vi "Main.vi"(6 "Folder names":string[](array[string])=["StaARx#[PLC]StaATesterRxSignals", "StaATx#[PLC]StaATesterTxSignals"], 8 "error in":errorcluster, 9 "Sequence Context":refnum<k7>, 11 "OPC UA In":refnum<class "Abstract.lvclass">=refnum) -> (0 "error out":errorcluster, 3 "OPC UA Out":refnum<class "Abstract.lvclass">)   [LabVIEW 2025, in "Abstract.lvclass"]
uses:
  Abstract.lvclass
  Tester Rx Dataset.ctl
  Tester Tx Dataset.ctl
  Abstract.lvclass/Abstract.ctl
  Read OPC UA Ref.vi
  Write Rx from PLC.vi
  Write Tx to PLC.vi
  Write Subscription.vi
  <vilib>/OPCUA/NI OPC UA Client.lvlib
panel:
  in  "Tx to PLC":T1
  out "Rx from PLC":T2={"Start"=FALSE, "NestStatus"=FALSE, "PalletID"=0, "BarcodeData"="P:10-000001R:04S:QMC2200001", "StepEcho"=0, "Cylinder_1"=FALSE, "Cylinder_2"=FALSE, "Cylinder_3"=FALSE, "Cylinder_4"=FALSE, "Cylinder_5"=FALSE, "ResultsAck"=FALSE, "Reset"=FALSE, "Stop"=FALSE, "FaultCode"=0}
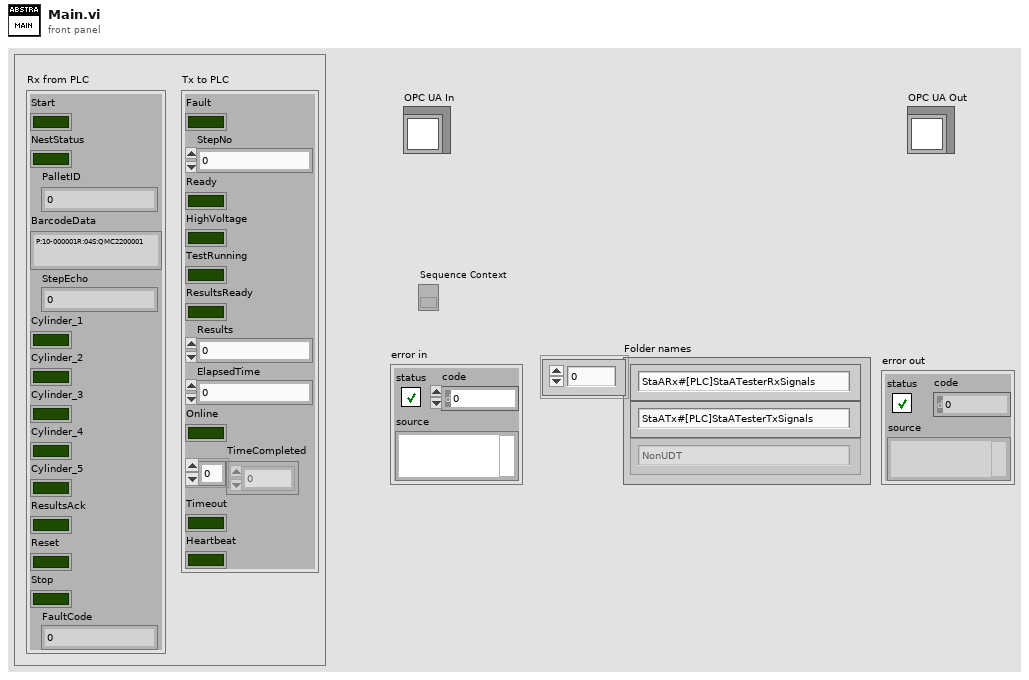
[diagram p1: front panel]
types:
  T1 = typedef "Abstract.lvclass/Tester Tx Dataset.ctl" = cluster{"Fault":bool, "StepNo":u32, "Ready":bool, "HighVoltage":bool, "TestRunning":bool, "ResultsReady":bool, "Results":u32, "ElapsedTime":u32, "Online":bool, "TimeCompleted":i32[], "Timeout":bool, "Heartbeat":bool}
  T2 = typedef "Abstract.lvclass/Tester Rx Dataset.ctl" = cluster{"Start":bool, "NestStatus":bool, "PalletID":u32, "BarcodeData":string, "StepEcho":u32, "Cylinder_1":bool, "Cylinder_2":bool, "Cylinder_3":bool, "Cylinder_4":bool, "Cylinder_5":bool, "ResultsAck":bool, "Reset":bool, "Stop":bool, "FaultCode":u32}
  T3 = typedef "OPC UA Client Refnum.ctl" = refnum<k21>
  T4 = typedef "Subscription ID.ctl" = u32
  T5 = cluster{"Event Registration Refnum":refnum<event-registration>, "Event Registration Refnum":refnum<event-registration>}
  T6 = typedef "TestStand - Status Monitor.ctl" = cluster{"Sequence Context":refnum<k7>, "Execution":refnum<k7>, "Termination Monitor":refnum<k7>}
  T7 = typedef "Subscription Data Change.ctl" = cluster{"node ID":T8, " value":variant, "timestamp":timestamp, "data type":T9, "status code":T10}
  T8 = typedef "NodeId.ctl" = string
  T9 = typedef "Data Type.ctl" = u16
  T10 = typedef "OPC UA StatusCode.ctl" = u32
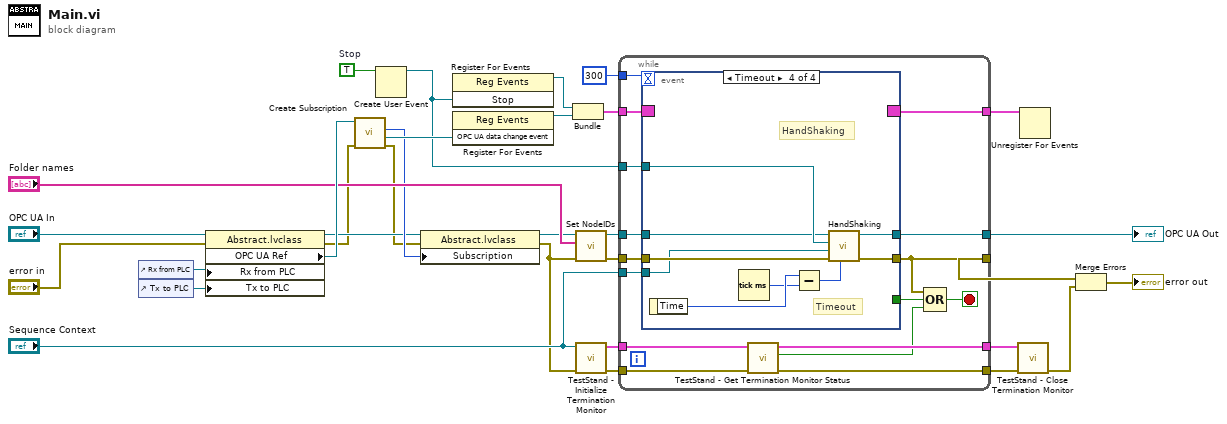
[diagram p0: block diagram]
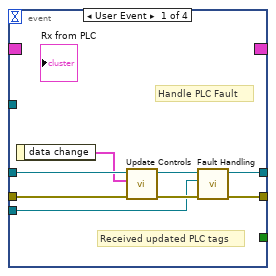
[diagram p2: hidden frame]
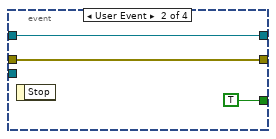
[diagram p3: hidden frame]
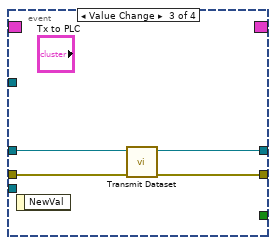
[diagram p4: hidden frame]
diagram:
  w19 = TRUE  # Stop
  n1 = control-ref of="Rx from PLC"() -> (w3:refnum<vi>)
  n2 = control-ref of="Tx to PLC"() -> (w2:refnum<vi>)
  n3 = property class="Abstract.lvclass"(reference="OPC UA In", error in="error in", "Rx from PLC"=w3, "Tx to PLC"=w2) -> (reference out=w10:refnum<class "Abstract.lvclass">, error out=w8:errorcluster, "OPC UA Ref"=w13:T3)
  n4 = call <vilib>:"Create Subscription.vi"("error in (no error)"=w8, "OPC UA client refnum in"=w13) -> ("error out"=w7:errorcluster, "OPC UA data change event"=w24:refnum<user-event>, "subscription ID out"=w11:T4)  [unwired: 5 in, 2 out]
  n5 = Create User Event(user event datatype=w19) -> (user event=w18:refnum<user-event>)  [unwired: 1 in, 1 out]
  n6 = property class="Abstract.lvclass"(reference=w10, error in=w7, "Subscription"=w11) -> (reference out=w5:refnum<class "Abstract.lvclass">, error out=w1:errorcluster)
  n7 = register-events(w18) -> (reference out=w20:refnum<event-registration>)  [unwired: 2 in, 1 out]
  n8 = register-events(w24) -> (reference out=w22:refnum<event-registration>)  [unwired: 2 in, 1 out]
  n9 = Bundle("Event Registration Refnum"=w20, "Event Registration Refnum"=w22) -> (w21:T5)  [unwired: 1 in]
  n10 = call "Set NodeIDs.vi"("error in (no error)"=w1, "PLC Folder Names"="Folder names", "AbstractUUT"=w5) -> ("error out"=w6:errorcluster, "AbstractUUT out"=w4:refnum<class "Abstract.lvclass">)  [unwired: 7 in]
  n11 = call <vilib>:"TestStand - Initialize Termination Monitor.vi"("error in (no error)"=w1, "Sequence Context In"="Sequence Context") -> ("error out"=w31:errorcluster, "Status Monitor Out"=w30:T6)  [unwired: 8 in]
  n12 = while {
    tunnel: w21 -> [w35]
    tunnel: w4 -> [w47]
    tunnel: w6 -> [w46]
    tunnel: [w37] -> w16
    tunnel: [w45] -> w27
    tunnel: w31 -> [w44]
    tunnel: w30 -> [w43]
    tunnel: [w41] -> w29
    tunnel: [w40] -> w28
    tunnel: [w39] -> w23
    tunnel: w18 -> [w34]
    tunnel: "Sequence Context" -> [w33]
    tunnel: 300 -> [w32]
    stop <- w42 stop-if-true
    n13 = event shown="[3] Timeout" {
      selector: w35 -> [_ _ _ _]
      dyn-events: [_ _ _ _] -> w45
      timeout: w32 -> [_ _ _ _]
      tunnel: w47 -> [w55 w58 w60 w65]
      tunnel: w46 -> [w54 w57 w61 w69]
      tunnel: [w52 w57 w62 w71] -> w37
      tunnel: [w51 w58 w59 w70] -> w39
      tunnel: [_ TRUE ("Stop") _ _] -> w36
      tunnel: w34 -> [_ _ _ w66]
      tunnel: w33 -> [w48 _ _ w64]
      event User Event {
        # "Handle PLC Fault"
        # "Received updated PLC tags"
        n14 = event-data() -> ("data change"=w49:T7[])  [unwired: 1 in]
        n15 = call "Update Controls.vi"("error in (no error)"=w54, "data change"=w49, "OPC UA in"=w55) -> ("error out"=w53:errorcluster, "OPC UA out"=w50:refnum<class "Abstract.lvclass">)  [unwired: 7 in]
        n16 = call "Fault Handling.vi"("error in (no error)"=w53, "Sequence Context"=w48, "OPC UA in"=w50) -> ("error out"=w52:errorcluster, "OPC UA out"=w51:refnum<class "Abstract.lvclass">)  [unwired: 7 in]
      }
      event User Event {
        n17 = event-data() -> ()  [unwired: 1 in, 1 out]
      }
      event Value Change {
        n18 = event-data() -> ()  [unwired: 1 in, 1 out]
        n19 = call "Transmit Dataset.vi"("error in (no error)"=w61, "OPC UA in"=w60) -> ("error out"=w62:errorcluster, "OPC UA out"=w59:refnum<class "Abstract.lvclass">)  [unwired: 8 in]
      }
      event Timeout {
        # "HandShaking"
        # "Timeout"
        n20 = event-data() -> ("Time"=w68:u32)  [unwired: 1 in]
        n21 = Tick Count (ms)() -> (millisecond timer value=w63:u32)
        n22 = Subtract(x=w68, y=w63) -> (x-y=w67:u32)
        n23 = call-dynamic "HandShaking.vi"("Elapsed Time"=w67, "error in (no error)"=w69, "Sequence Context"=w64, "Stop"=w66, "OPC UA in"=w65) -> ("error out"=w71:errorcluster, "OPC UA out"=w70:refnum<class "Abstract.lvclass">)  [unwired: 5 in]
      }
    }
    n24 = call <vilib>:"TestStand - Get Termination Monitor Status.vi"("error in (no error)"=w44, "Status Monitor In"=w43) -> ("error out"=w41:errorcluster, "Terminating or Aborting"=w38:bool, "Status Monitor Out"=w40:T6)  [unwired: 7 in]
    n25 = Compound Arithmetic op=OR(w37, w36, w38) -> (w42:bool)
  }
  "OPC UA Out" <- w23
  n26 = call <vilib>:"TestStand - Close Termination Monitor.vi"("error in (no error)"=w29, "Status Monitor In"=w28) -> ("error out"=w25:errorcluster)  [unwired: 9 in]
  n27 = Unregister For Events(event registration refnum=w27) -> ()  [unwired: 1 in, 1 out]
  n28 = Merge Errors(w16, w25) -> (→"error out":errorcluster)
